vi "Start.vi"(8 "error in (no error)":errorcluster, 9 "Timeout [ms] (-1)":i32=-1, 11 "Process In":refnum<class "Process.lvclass">) -> (0 "error out":errorcluster, 1 "timed out?":bool, 3 "Process Out":refnum<class "Process.lvclass">)   [LabVIEW 2020, in "Process.lvclass"]
doc: "This VI starts the process which runs asyncronously. The VI blocks the execution until the process has reached its' running state, or the specified timeout expires."
uses:
  Process.lvclass
  Process.lvclass/Process.ctl
  <vilib>/ErrorRing/Error Ring.xnode
  <vilib>/Utility/error.llb/Error Cluster From Error Code.vi
  Public/Lifecycle/Lifecycle State.ctl
  Logging/Logging.lvclass
  C:/git/astemes-triarc-framework/source/Framework/Logging/Logging.lvclass
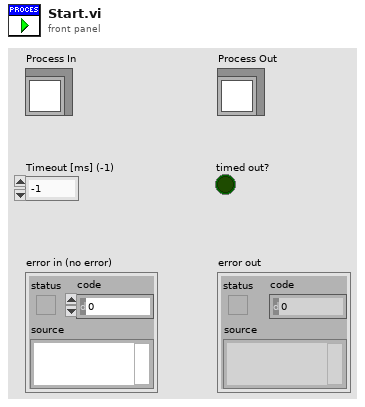
[diagram p1: front panel]
types:
  T1 = typedef "Process.lvclass/Lifecycle State.ctl" = enum16{"Uninitialized", "Initialized", "Started", "Running", "Stopped", "Finished"}
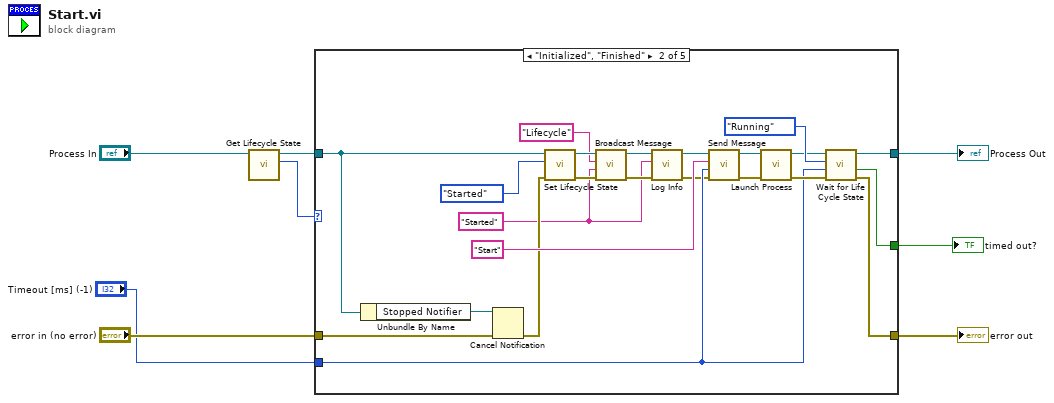
[diagram p0: block diagram]
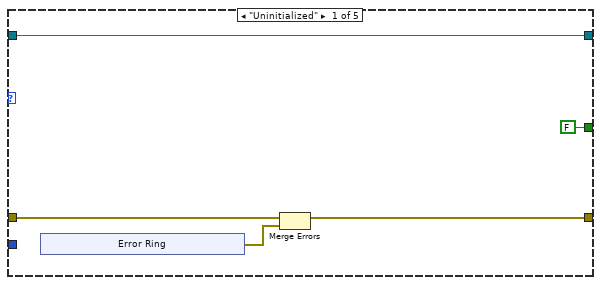
[diagram p2: hidden frame]
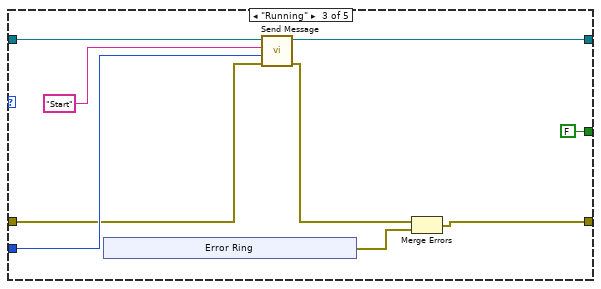
[diagram p3: hidden frame]
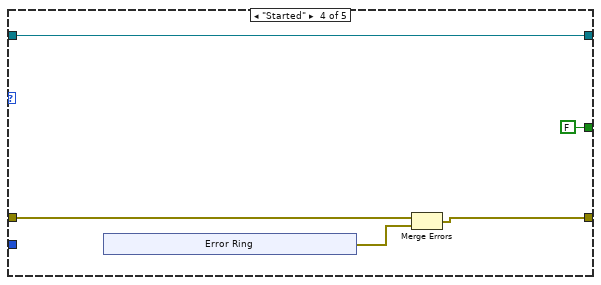
[diagram p4: hidden frame]
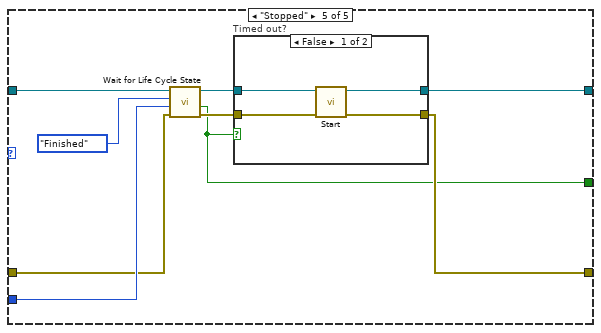
[diagram p5: hidden frame]
diagram:
  n1 = call "Get Lifecycle State.vi"("Process In"="Process In") -> ("Lifecycle State"=w2:T1, "Process Out"=w3:refnum<class "Process.lvclass">)  [unwired: 7 in, 2 out]
  n2 = case shown="\"Initialized\", \"Finished\"" w2 {
    tunnel: [w12 w35 w46 w58 w64] -> w7
    tunnel: [w11 w34 w48 w56 w66] -> w6
    tunnel: w3 -> [w12 w38 w45 w58 w71]
    tunnel: "error in (no error)" -> [w10 w39 w41 w55 w68]
    tunnel: "Timeout [ms] (-1)" -> [_ w25 w43 _ w69]
    tunnel: [FALSE ("timed out?") w24 FALSE ("timed out?") FALSE ("timed out?") w63] -> w1
    frame "Uninitialized" {
      n3 = xnode "Error Ring"() -> ("error out"=w13:errorcluster)
      n4 = Merge Errors(w10, w13) -> (w11:errorcluster)
    }
    frame "Initialized", "Finished" {
      w18 = "Started" ("Message")
      n5 = Unbundle By Name(w38) -> ("Stopped Notifier"=w40:refnum<notifier>)
      n6 = Cancel Notification(0:w40, 3:w39) -> (11:w32:errorcluster)  [unwired: 2 out]
      n7 = call "Set Lifecycle State.vi"("error in (no error)"=w32, "Lifecycle State"=Lifecycle_State."Started", "Process In"=w38) -> ("error out"=w30:errorcluster, "Process Out"=w28:refnum<class "Process.lvclass">)  [unwired: 7 in]
      n8 = call-dynamic "Broadcast Message.vi"("error in (no error)"=w30, "Message Data"=w18, "Message"="Lifecycle", "Process In"=w28) -> ("error out"=w29:errorcluster, "Process Out"=w20:refnum<class "Process.lvclass">)  [unwired: 6 in]
      n9 = call "Log Info.vi"("error in (no error)"=w29, "Message"=w18, "Logging In"=w20) -> ("error out"=w21:errorcluster, "Logging Out"=w19:refnum<class "Process.lvclass">)  [unwired: 7 in]
      n10 = call "Send Message.vi"("error in (no error)"=w21, "Message Data"=w25, "Message"="Start", "Process In"=w19) -> ("error out"=w37:errorcluster, "Process Out"=w23:refnum<class "Process.lvclass">)  [unwired: 6 in]
      n11 = call "Launch Process.vi"("error in (no error)"=w37, "Process in"=w23) -> ("error out"=w31:errorcluster, "Process out"=w22:refnum<class "Process.lvclass">)  [unwired: 8 in]
      n12 = call "Wait for Life Cycle State.vi"("error in (no error)"=w31, "timeout in ms (-1)"=w25, "Lifecycle State"=Lifecycle_State."Running", "Process In"=w22) -> ("error out"=w34:errorcluster, "timed out?"=w24:bool, "Process Out"=w35:refnum<class "Process.lvclass">)  [unwired: 5 in]
    }
    frame "Running" {
      n13 = xnode "Error Ring"() -> ("error out"=w49:errorcluster)
      n14 = call "Send Message.vi"("error in (no error)"=w41, "Message Data"=w43, "Message"="Start", "Process In"=w45) -> ("error out"=w42:errorcluster, "Process Out"=w46:refnum<class "Process.lvclass">)  [unwired: 6 in]
      n15 = Merge Errors(w42, w49) -> (w48:errorcluster)
    }
    frame "Started" {
      n16 = xnode "Error Ring"() -> ("error out"=w57:errorcluster)
      n17 = Merge Errors(w55, w57) -> (w56:errorcluster)
    }
    frame "Stopped" {
      n18 = call "Wait for Life Cycle State.vi"("error in (no error)"=w68, "timeout in ms (-1)"=w69, "Lifecycle State"=Lifecycle_State."Finished", "Process In"=w71) -> ("error out"=w67:errorcluster, "timed out?"=w63:bool, "Process Out"=w65:refnum<class "Process.lvclass">)  [unwired: 5 in]
      n19 = case "Timed out?" shown="False" w63 {
        tunnel: w67 -> [w75 w76]
        tunnel: [w74 w76] -> w66
        tunnel: w65 -> [w73 w77]
        tunnel: [w72 w77] -> w64
        frame False {
          n20 = call "Start.vi"("error in (no error)"=w75, "Process In"=w73) -> ("error out"=w74:errorcluster, "Process Out"=w72:refnum<class "Process.lvclass">)  [unwired: 7 in, 1 out]
        }
        frame True {
        }
      }
    }
  }
  "error out" <- w6
  "Process Out" <- w7
  "timed out?" <- w1
